vi "Show Toast Notification.vi"(8 "error in":errorcluster, 10 "Toast Notification":refnum<k24>, 11 "Toast Notifier in":refnum<k24>) -> (0 "error out":errorcluster, 3 "Toast Notifier out":refnum<k24>)   [LabVIEW 2026, in "ToastNotification.lvlib" / "Toast Native.lvlib"]
doc: "Display a borrowed Toast Notification through ToastNotifierCompat.Show. Can display a Windows notification. Skipped on incoming error. Toast Notifier out aliases its input. Does not close either borrowed object or register callbacks. Release only temporary invocation results and metadata. Caller closes notifier, notification and document after their final use."
uses:
  Toast Native.lvlib
  Reflection DotNet/Reflection DotNet.lvlib
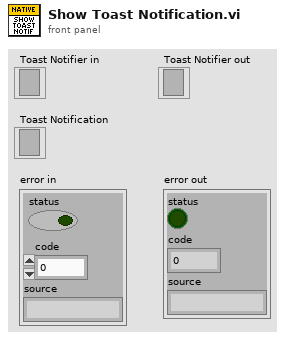
[diagram p1: front panel]
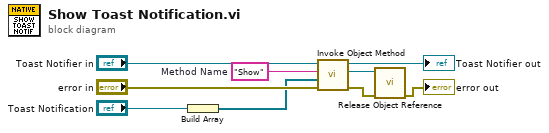
[diagram p0: block diagram]
diagram:
  w7 = "Show"  # Method Name
  n1 = Build Array("Toast Notification") -> (w5:refnum<k24>[])
  n2 = call "Invoke Object Method.vi"("error in"="error in", "parameters"=w5, "Method Name"=w7, "Object in"="Toast Notifier in") -> ("error out"=w3:errorcluster, "Return Value"=w1:refnum<k24>, "Object out"=→"Toast Notifier out":refnum<k24>)  [unwired: 5 in]
  n3 = call "Release Object Reference.vi"("error in"=w3, "object"=w1) -> ("error out"=→"error out":errorcluster)  [unwired: 9 in]
